vi "HostMem_Probe.vi"(11 "OpenLvVision_OpenCv.lvlib:HostMem":refnum<class "HostMem.lvclass">) -> (2 "Value String":string, 3 "Pause VI":bool)   [LabVIEW 2020, in "OpenLvVision_OpenCv.lvlib" / "Cuda.lvlib" / "HostMem.lvclass"]
uses:
  HostMem.lvclass
  C:/Users/lukas/Downloads/OpenLvVision_OpenCv/SourceCode/LabView/OpenLvVision_OpenCv/_LvHelpers/EdvrObject/EdvrObject.lvclass
  TypeDef/HostMatInfo.ctl
  TypeDef/cvType.ctl
  _LvHelpers/EdvrObject/EdvrObject.lvclass/EdvrObject.ctl
  <vilib>/OpenLvVision/OpenLvVision_Image/Management/TypeDef/OLV ImageType.ctl
  CopyToArray/HostMem CopyToArray_2D-U8.vi
  CopyToArray/HostMem CopyToArray_2D-I8.vi
  CopyToArray/HostMem CopyToArray_2D-U16.vi
  CopyToArray/HostMem CopyToArray_2D-I16.vi
  CopyToArray/HostMem CopyToArray_2D-I32.vi
  CopyToArray/HostMem CopyToArray_2D-SGL.vi
  CopyToArray/HostMem CopyToArray_2D-DBL.vi
  CopyToArray/HostMem CopyToArray_2D-ColorU32.vi
  CopyToArray/HostMem CopyToArray_2D-ColorU64.vi
  CopyToArray/HostMem CopyToArray_2D-CSG.vi
  CopyToArray/HostMem CopyToArray_2D-CDB.vi
  _LvHelpers/EdvrObject/EdvrObject.lvclass
  <vilib>/OpenLvVision/OpenLvVision_Image/Management/OLV Management.lvlib
  OpenLvVision_OpenCv.lvlib
panel:
  in  "Probe Type":enum16{"Array", "Image"}(ring)
  out "HostMatInfo":T1
  out "Reference":u64 format="%.0x"
  out "Tab Control":enum32{"Array", "Image"}(tab)
  out "Array":T3(tab)
  out "CV_8UC1":u8[][](array[numeric])
  out "CV_8SC1":i8[][](array[numeric])
  out "CV_16UC1":u16[][](array[numeric])
  out "CV_16SC1":i16[][](array[numeric])
  out "CV_32SC1":i32[][](array[numeric])
  out "CV_32FC1":sgl[][](array[numeric])
  out "CV_64FC1":dbl[][](array[numeric])
  out "CV_8UC4":u32[][](array[numeric])
  out "CV_16UC4":u64[][](array[numeric])
  out "CV_32FC2":csg[][](array[numeric])
  out "CV_64FC2":cdb[][](array[numeric])
  out "Image":T4(plugin-control)
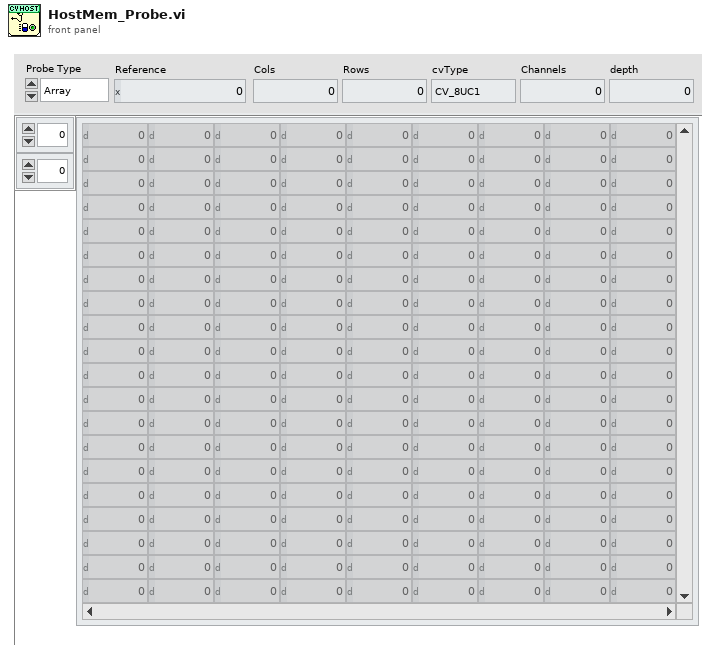
[diagram p1: front panel]
types:
  T1 = typedef "OpenLvVision_OpenCv.lvlib/HostMatInfo.ctl" = cluster{"Rows":i32, "Cols":i32, "cvType":T2, "Channels":i32, "depth":i32}
  T2 = typedef "OpenLvVision_OpenCv.lvlib/cvType.ctl" = enum32{"CV_8UC1", "CV_8SC1", "CV_16UC1", "CV_16SC1", "CV_32SC1", "CV_32FC1", "CV_64FC1", "CV_16FC1", "CV_8UC2", "CV_8SC2", "CV_16UC2", "CV_16SC2", "CV_32SC2", "CV_32FC2", "CV_64FC2", "CV_16FC2", "CV_8UC3", "CV_8SC3", "CV_16UC3", "CV_16SC3", "CV_32SC3", "CV_32FC3", "CV_64FC3", "CV_16FC3", "CV_8UC4", "CV_8SC4", "CV_16UC4", "CV_16SC4", "CV_32SC4", "CV_32FC4", "CV_64FC4", "CV_16FC4"}
  T3 = enum32{"CV_8UC1", "CV_8SC1", "CV_16UC1", "CV_16SC1", "CV_32SC1", "CV_32FC1", "CV_64FC1", "NotSupported", "CV_8UC4", "CV_16UC4", "CV_32FC2", "CV_64FC2"}
  T4 = typedef "IMAQ Image.ctl" = refnum<image>
  T5 = typedef "OpenLvVision_OpenCv.lvlib/EdvrObject.lvclass/Edvr.ctl" = refnum<data-value>
  T6 = typedef "OLV OpenLvVision_Image.lvlib/OLV Management.lvlib/OLV ImageType.ctl" = enum16{"Mono U8", "Mono U16", "Mono I16", "Mono SGL", "Color U32", "Color U64", "Complex CSG"}
  T7 = typedef "OLV OpenLvVision_Image.lvlib/OLV Management.lvlib/OLV Image.ctl" = refnum<image>
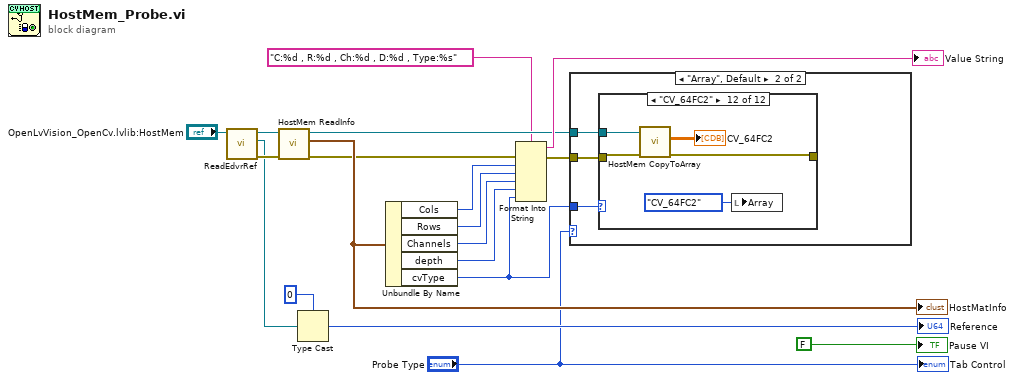
[diagram p0: block diagram]
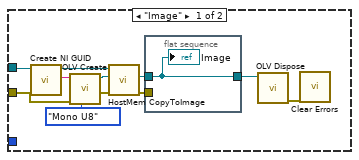
[diagram p2: hidden frame]
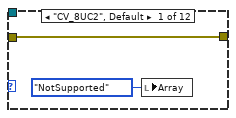
[diagram p3: hidden frame]
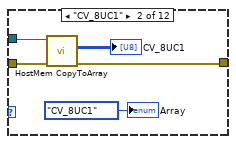
[diagram p4: hidden frame]
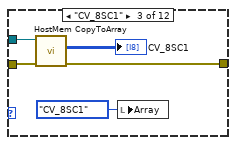
[diagram p5: hidden frame]
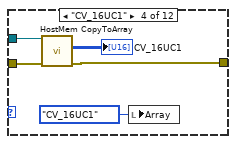
[diagram p6: hidden frame]
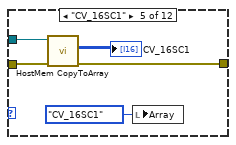
[diagram p7: hidden frame]
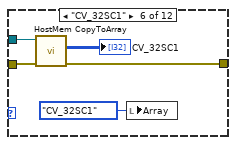
[diagram p8: hidden frame]
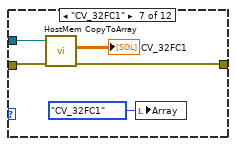
[diagram p9: hidden frame]
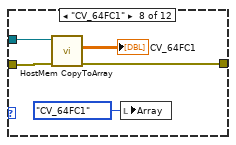
[diagram p10: hidden frame]
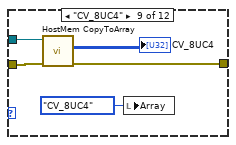
[diagram p11: hidden frame]
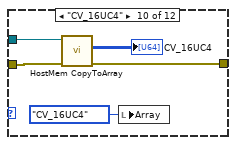
[diagram p12: hidden frame]
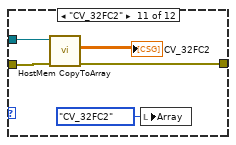
[diagram p13: hidden frame]
diagram:
  n1 = call "ReadEdvrRef.vi"("EdvrObject in"="OpenLvVision_OpenCv.lvlib:HostMem") -> ("error out"=w16:errorcluster, "Edvr"=w15:T5, "EdvrObject out"=w4:refnum<class "HostMem.lvclass">)  [unwired: 8 in]
  n2 = call "HostMem ReadInfo.vi"("error in (no error)"=w16, "HostMem in"=w4) -> ("error out"=w13:errorcluster, "HostMatInfo"=w14:T1, "HostMem out"=w6:refnum<class "HostMem.lvclass">)  [unwired: 7 in]
  "HostMatInfo" <- w14
  n3 = Type Cast(type=u64 0, x=w15) -> (*(type *) &x=→"Reference":u64)
  n4 = Unbundle By Name(w14) -> ("Cols"=w12:i32, "Rows"=w11:i32, "Channels"=w10:i32, "depth"=w9:i32, "cvType"=w2:T2)
  n5 = Format Into String(format string="C:%d , R:%d , Ch:%d , D:%d , Type:%s", error in=w13, w12, w11, w10, w9, w2) -> (resulting string=→"Value String":string, error out=w7:errorcluster)  [unwired: 1 in]
  n6 = case shown="\"Array\", Default" "Probe Type" {
    tunnel: w7 -> [w27 w33]
    tunnel: w6 -> [w28 w32]
    tunnel: w2 -> [_ w31]
    frame "Image" {
      n7 = call <vilib>:"Create NI GUID.vi"() -> ("NI GUID"=w24:string)
      n8 = call <vilib>:"OLV Create.vi"("Image Type"=OLV_ImageType."Mono U8", "error in"=w27, "Image Name"=w24) -> ("error out"=w26:errorcluster, "Image Reference Out"=w25:T7)  [unwired: 7 in]
      n9 = call "HostMem CopyToImage.vi"("error in (no error)"=w26, "Dst"=w25, "HostMem in"=w28) -> ("error out"=w22:errorcluster, "Dst out"=w29:T4)  [unwired: 6 in, 1 out]
      n10 = flat-sequence {
        tunnel: w29 -> [w30]
        tunnel: w22 -> [_]
        tunnel: [w30] -> w21
        frame #0 {
          "Image" <- w30
        }
      }
      n11 = call <vilib>:"OLV Dispose.vi"("Image Reference In"=w21) -> ("error out"=w20:errorcluster)  [unwired: 10 in]
      n12 = call <vilib>:"Clear Errors.vi"("error in (no error)"=w20) -> ()  [unwired: 5 in, 2 out]
    }
    frame "Array", Default {
      n13 = case shown="\"CV_64FC2\"" w31 {
        tunnel: w33 -> [w34 w38 w43 w48 w53 w59 w63 w69 w74 w79 w84 w88]
        tunnel: w32 -> [_ w39 w44 w49 w54 w58 w64 w68 w73 w78 w83 w89]
        tunnel: [w34 w36 w41 w46 w51 w56 w61 w67 w72 w76 w81 w86] -> _
        frame "CV_8UC2", Default {
          n14 = local write "Array"(T3."NotSupported" ("Array")) -> ()
        }
        frame "CV_8UC1" {
          n15 = call-poly "HostMem CopyToArray.vi"("error in (no error)"=w38, "HostMem in"=w39) -> ("error out"=w36:errorcluster, "Array"=→"CV_8UC1":u8[][])  [unwired: 7 in, 1 out]
          "Array" <- T3."CV_8UC1" ("Array")
        }
        frame "CV_8SC1" {
          n16 = call-poly "HostMem CopyToArray.vi"("error in (no error)"=w43, "HostMem in"=w44) -> ("error out"=w41:errorcluster, "Array"=→"CV_8SC1":i8[][])  [unwired: 7 in, 1 out]
          n17 = local write "Array"(T3."CV_8SC1" ("Array")) -> ()
        }
        frame "CV_16UC1" {
          n18 = call-poly "HostMem CopyToArray.vi"("error in (no error)"=w48, "HostMem in"=w49) -> ("error out"=w46:errorcluster, "Array"=→"CV_16UC1":u16[][])  [unwired: 7 in, 1 out]
          n19 = local write "Array"(T3."CV_16UC1" ("Array")) -> ()
        }
        frame "CV_16SC1" {
          n20 = call-poly "HostMem CopyToArray.vi"("error in (no error)"=w53, "HostMem in"=w54) -> ("error out"=w51:errorcluster, "Array"=→"CV_16SC1":i16[][])  [unwired: 7 in, 1 out]
          n21 = local write "Array"(T3."CV_16SC1" ("Array")) -> ()
        }
        frame "CV_32SC1" {
          n22 = call-poly "HostMem CopyToArray.vi"("error in (no error)"=w59, "HostMem in"=w58) -> ("error out"=w56:errorcluster, "Array"=→"CV_32SC1":i32[][])  [unwired: 7 in, 1 out]
          n23 = local write "Array"(T3."CV_32SC1" ("Array")) -> ()
        }
        frame "CV_32FC1" {
          n24 = call-poly "HostMem CopyToArray.vi"("error in (no error)"=w63, "HostMem in"=w64) -> ("error out"=w61:errorcluster, "Array"=→"CV_32FC1":sgl[][])  [unwired: 7 in, 1 out]
          n25 = local write "Array"(T3."CV_32FC1" ("Array")) -> ()
        }
        frame "CV_64FC1" {
          n26 = call-poly "HostMem CopyToArray.vi"("error in (no error)"=w69, "HostMem in"=w68) -> ("error out"=w67:errorcluster, "Array"=→"CV_64FC1":dbl[][])  [unwired: 7 in, 1 out]
          n27 = local write "Array"(T3."CV_64FC1" ("Array")) -> ()
        }
        frame "CV_8UC4" {
          n28 = call-poly "HostMem CopyToArray.vi"("error in (no error)"=w74, "HostMem in"=w73) -> ("error out"=w72:errorcluster, "Array"=→"CV_8UC4":u32[][])  [unwired: 7 in, 1 out]
          n29 = local write "Array"(T3."CV_8UC4" ("Array")) -> ()
        }
        frame "CV_16UC4" {
          n30 = call-poly "HostMem CopyToArray.vi"("error in (no error)"=w79, "HostMem in"=w78) -> ("error out"=w76:errorcluster, "Array"=→"CV_16UC4":u64[][])  [unwired: 7 in, 1 out]
          n31 = local write "Array"(T3."CV_16UC4" ("Array")) -> ()
        }
        frame "CV_32FC2" {
          n32 = call-poly "HostMem CopyToArray.vi"("error in (no error)"=w84, "HostMem in"=w83) -> ("error out"=w81:errorcluster, "Array"=→"CV_32FC2":csg[][])  [unwired: 7 in, 1 out]
          n33 = local write "Array"(T3."CV_32FC2" ("Array")) -> ()
        }
        frame "CV_64FC2" {
          n34 = call-poly "HostMem CopyToArray.vi"("error in (no error)"=w88, "HostMem in"=w89) -> ("error out"=w86:errorcluster, "Array"=→"CV_64FC2":cdb[][])  [unwired: 7 in, 1 out]
          n35 = local write "Array"(T3."CV_64FC2" ("Array")) -> ()
        }
      }
    }
  }
  "Pause VI" <- FALSE
  "Tab Control" <- "Probe Type"
